vi "Create Value - 1D Array String.vi"(8 "error in (no error)":errorcluster, 9 "Create as 1D Array?":bool=TRUE, 10 "1D String":string[](array[string])) -> (0 "error out":errorcluster, 3 "JSON Tree":variant)   [LabVIEW 2014, in "i3-json.lvlib"]
doc: "Creates a new JSON Object of the given type"
uses:
  i3-json.lvlib
  JSON Types/JSON Type.ctl
  JSON Types/JSON Compatible Type.ctl
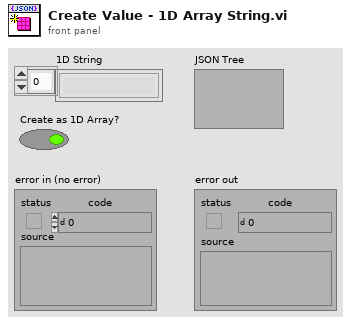
[diagram p1: front panel]
types:
  T1 = typedef "i3-json.lvlib/JSON Compatible Type.ctl" = enum16{"1D Double Array", "1D String Array", "1D Boolean Array", "Unknown"}
  T2 = typedef "i3-json.lvlib/JSON Type.ctl" = enum8{"JSON Compatible", "JSON Array", "JSON Object", "JSON Null", "Double", "String", "Boolean", "Unknown"}
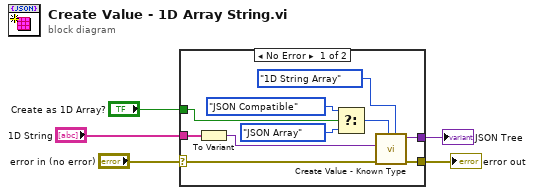
[diagram p0: block diagram]
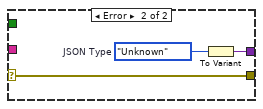
[diagram p2: hidden frame]
diagram:
  n1 = case shown="No Error" "error in (no error)" {
    selector: "error in (no error)" -> [w14 w16]
    tunnel: [w13 w16] -> w4
    tunnel: [w15 w17] -> w3
    tunnel: "Create as 1D Array?" -> [w7 _]
    tunnel: "1D String" -> [w6 _]
    frame No Error {
      n2 = To Variant(anything=w6) -> (Variant=w12:variant)
      n3 = Select(t=JSON_Type."JSON Compatible" ("JSON Type"), s=w7, f=JSON_Type."JSON Array" ("JSON Type")) -> (s? t:f=w9:T2)
      n4 = call "Create Value - Known Type.vi"("JSON Compatible Type"=JSON_Compatible_Type."1D String Array", "JSON Type"=w9, "error in (no error)"=w14, "Value"=w12) -> ("error out"=w13:errorcluster, "JSON Tree"=w15:variant)  [unwired: 6 in]
    }
    frame Error {
      w18 = JSON_Type."Unknown"  # JSON Type
      n5 = To Variant(anything=w18) -> (Variant=w17:variant)
    }
  }
  "JSON Tree" <- w3
  "error out" <- w4
